vi "DriverStation Are Outputs Enabled.vi"(8 "error in":errorcluster) -> (0 "error out":errorcluster, 3 "OutputsEnabled?":bool)   [LabVIEW 2023, in "MrcLib.lvlib"]
doc: "Are actuators and output I/O enabled. Outputs will be disabled due to loss of communications, overvoltage or brownout conditions on the input power to the robot controller."
uses:
  <vilib>/MRC/MrcLib.lvlib
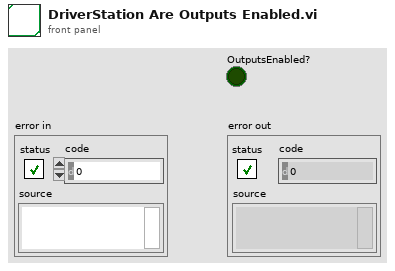
[diagram p1: front panel]
types:
  T1 = typedef "MrcLib.lvlib/MRC_ControlData.ctl" = cluster{"controlFlags":u32, "matchTime":u16, "currentOpMode":u64, "gameDataLength":u8, "game data":T2}
  T2 = typedef "MRC Str64.ctl" = cluster{"[0]":u8, "[1]":u8, "[2]":u8, "[3]":u8, "[4]":u8, "[5]":u8, "[6]":u8, "[7]":u8, "[8]":u8, "[9]":u8, "[10]":u8, "[11]":u8, "[12]":u8, "[13]":u8, "[14]":u8, "[15]":u8, "[16]":u8, "[17]":u8, "[18]":u8, "[19]":u8, "[20]":u8, "[21]":u8, "[22]":u8, "[23]":u8, "[24]":u8, "[25]":u8, "[26]":u8, "[27]":u8, "[28]":u8, "[29]":u8, "[30]":u8, "[31]":u8, "[32]":u8, "[33]":u8, "[34]":u8, "[35]":u8, "[36]":u8, "[37]":u8, "[38]":u8, "[39]":u8, "[40]":u8, "[41]":u8, "[42]":u8, "[43]":u8, "[44]":u8, "[45]":u8, "[46]":u8, "[47]":u8, "[48]":u8, "[49]":u8, "[50]":u8, "[51]":u8, "[52]":u8, "[53]":u8, "[54]":u8, "[55]":u8, "[56]":u8, "[57]":u8, "[58]":u8, "[59]":u8, "[60]":u8, "[61]":u8, "[62]":u8, "[63]":u8}
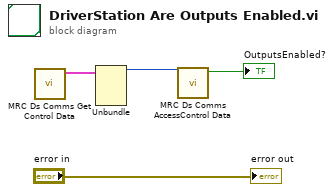
[diagram p0: block diagram]
diagram:
  n1 = call <vilib>:"MRC Ds Comms Get Control Data.vi"() -> ("data out"=w3:T1)  [unwired: 10 in, 1 out]
  n2 = Unbundle(w3) -> ("controlFlags"=w2:u32)  [unwired: 4 out]
  n3 = call <vilib>:"MRC Ds Comms AccessControl Data.vi"("controlFlag"=w2) -> ("Enabled"=→"OutputsEnabled?":bool)  [unwired: 7 in, 3 out]
  "error out" <- "error in"
